vi "Simple SCP File Download.vi"() -> ()   [LabVIEW 2018]
doc: "Downloads, or receives, a relatively small file from a remote SSH server. This is similar to the SCP command line utility when transferring, or copying, a remote file to a local destination. If performance is poor or memory is limited on the local machine, then it could be because the file is relatively large and this implementation is not very efficient for relatively large files."
uses:
  Toolkit/Session/Support/Create from SSH.vi
  Toolkit/Session/Support/Password Authentication.vi
  Toolkit/Channel/Support/Create from SCP Receive.vi
  Toolkit/Channel/Support/Destroy to Session.vi
  Toolkit/Session/Support/Destroy to SSH.vi
  Toolkit/SSH/SSH.lvclass
  Toolkit/Session/Session.lvclass
  Toolkit/Channel/Channel.lvclass
panel:
  in  "Remote File":string
  in  "Local File":path
  in  "Remote SSH Server":string
  in  "Password":string
  in  "Username":string
  # "Overview: Demonstrates transferring, or downloading, a remote file from a SSH server, similar to the SCP command line utility\nInstructions:\n1. Enter the IP address or host name of the remote SSH server. This can be a CompactRIO (cRIO) running the National Instruments Linux Real-Time (NI Linux RT) operating system with the Enable Secure Shell Server (sshd) checkbox checked. \n2. Enter a username. If using a cRIO with a default configuration, then the username is \"admin\".\n3. Enter a password for the username. If using a cRIO with a default configuration, then the password is blank (empty).\n4. Enter the path and/or filename of the remote file to download. Typically, this is a POSIX/UNIX file path with a backslash, \"/\", use to separate directories and the default directory is the remote user's home directory, i.e. \"/home/admin\" on a default configured cRIO.\n5. Select a destination on the local computer for the transfer/download from the remote SSH server.\n6. Run this VI."
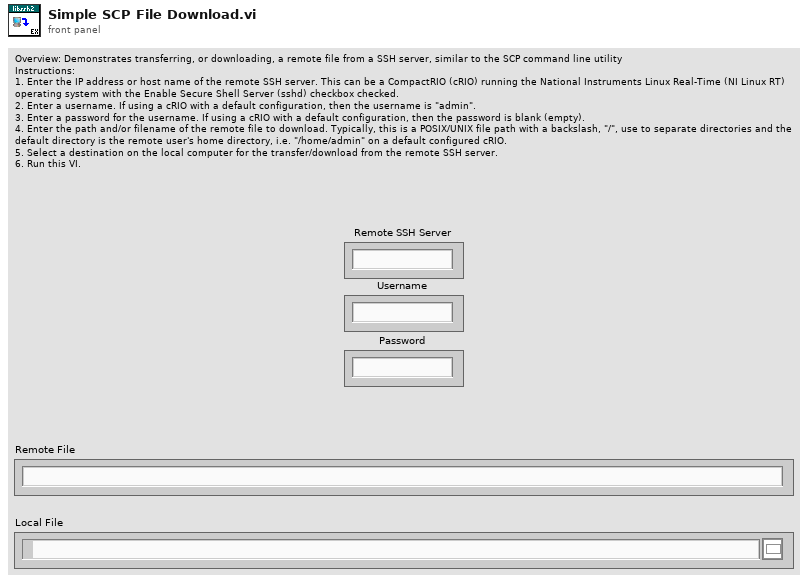
[diagram p1: front panel]
types:
  T1 = enum16{"open", "replace", "create", "open or create", "replace or create", "replace or create with confirmation"}
  T2 = typedef "Toolkit.lvlib/Permissions.ctl" = cluster{"Owner":T3, "Group":T3, "Others":T3}
  T3 = typedef "Toolkit.lvlib/Modes.ctl" = cluster{"Read":bool, "Write":bool, "Execute":bool}
  T4 = cluster{"Access Time":u64, "File Size":u64, "Modified Time":u64, "Permissions":T2}
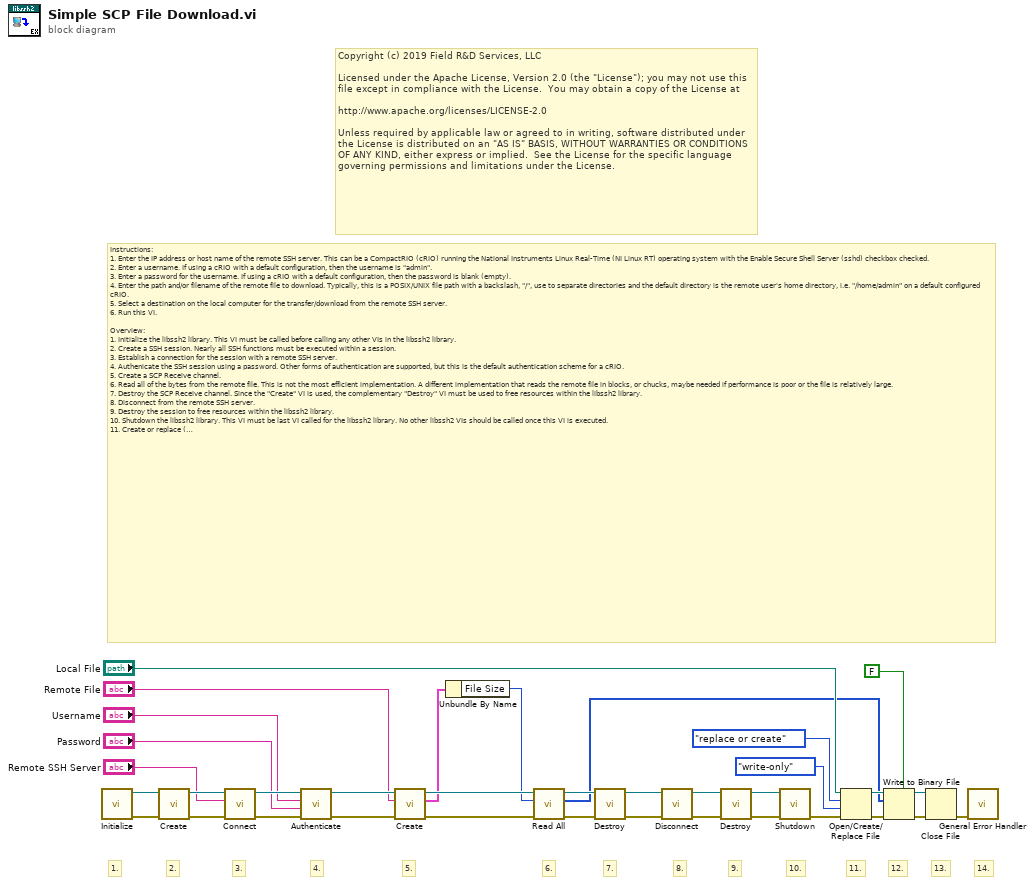
[diagram p0: block diagram]
diagram:
  # "Copyright (c) 2019 Field R&D Services, LLC\n\nLicensed under the Apache License, Version 2.0 (the \"License\"); you may not use this file except in compliance with the License.  You may obtain a copy of the License at\n\nhttp://www.apache.org/licenses/LICENSE-2.0\n\nUnless required by applicable law or agreed to in writing, software distributed under the License is distributed on an \"AS IS\" BASIS, WITHOUT WARRANTIES OR CONDITIONS OF ANY KIND, either express or implied.  See the License for the specific language governing permissions and limitations under the License."
  # "14."
  # "13."
  # "12."
  # "11."
  # "10."
  # "9."
  # "8."
  # "7."
  # "6."
  # "5."
  # "4."
  # "3."
  # "2."
  # "1."
  # "Instructions:\n1. Enter the IP address or host name of the remote SSH server. This can be a CompactRIO (cRIO) running the National Instruments Linux Real-Time (NI Linux RT) operating system with the Enable Secure Shell Server (sshd) checkbox checked. \n2. Enter a username. If using a cRIO with a default configuration, then the username is \"admin\".\n3. Enter a password for the username. If using a cRIO with a default configuration, then the password is blank (empty).\n4. Enter the path and/or filename of the remote file to download. Typically, this is a POSIX/UNIX file path with a backslash, \"/\", use to separate directories and the default directory is the remote user's home directory, i.e. \"/home/admin\" on a default configured cRIO.\n5. Select a destination on the local computer for the transfer/download from the remote SSH server.\n6. Run this VI.\n\nOverview:\n1. Initialize the libssh2 library. This VI must be called before calling any other VIs in the libssh2 library.\n2. Create a SSH session. Nearly all SSH functions must be executed within a session.\n3. Establish a connection for the session with a remote SSH server.\n4. Authenicate the SSH session using a password. Other forms of authentication are supported, but this is the default authentication scheme for a cRIO. \n5. Create a SCP Receive channel.\n6. Read all of the bytes from the remote file. This is not the most efficient implementation. A different implementation that reads the remote file in blocks, or chucks, maybe needed if performance is poor or the file is relatively large.\n7. Destroy the SCP Receive channel. Since the \"Create\" VI is used, the complementary \"Destroy\" VI must be used to free resources within the libssh2 library.\n8. Disconnect from the remote SSH server.\n9. Destroy the session to free resources within the libssh2 library.\n10. Shutdown the libssh2 library. This VI must be last VI called for the libssh2 library. No other libssh2 VIs should be called once this VI is executed.\n11. Create or replace (overwrite) a file to write the read contents from the remote file.\n12. Write the data from the remote file.\n13. Close the file. This is not strictly necessary, but it is good practice.\n14. Provide some error handling and reporting. Libssh2 errors will be in the -8100 range."
  n1 = call "Initialize.vi"() -> ("Error Out"=w22:errorcluster, "SSH"=w21:refnum<class "SSH.lvclass">)  [unwired: 10 in]
  n2 = call-poly "Create.vi"("Error In"=w22, "SSH"=w21) -> ("Error Out"=w34:errorcluster, "Sesssion"=w35:refnum<class "Session.lvclass">)  [unwired: 8 in]
  n3 = call "Connect.vi"("Error In"=w34, "Address"="Remote SSH Server", "Session In"=w35) -> ("Error Out"=w32:errorcluster, "Sesssion Out"=w33:refnum<class "Session.lvclass">)  [unwired: 7 in]
  n4 = call-poly "Authenticate.vi"("Error In"=w32, "Password"="Password", "Username"="Username", "Session In"=w33) -> ("Error Out"=w19:errorcluster, "Sesssion Out"=w20:refnum<class "Session.lvclass">)  [unwired: 6 in]
  n5 = call-poly "Create.vi"("Error In"=w19, "Remote Source Path"="Remote File", "Session"=w20) -> ("Error Out"=w4:errorcluster, "File Information"=w3:T4, "Channel"=w5:refnum<class "Channel.lvclass">)  [unwired: 6 in]
  n6 = Unbundle By Name(w3) -> ("File Size"=w2:u64)
  n7 = call "Read All.vi"("Error In"=w4, "Max Read Size"=w2, "Channel In"=w5) -> ("Error Out"=w9:errorcluster, "Data"=w7:u8[], "Channel Out"=w8:refnum<class "Channel.lvclass">)  [unwired: 5 in, 1 out]
  n8 = call-poly "Destroy.vi"("Error In"=w9, "Channel"=w8) -> ("Error Out"=w27:errorcluster, "Session"=w28:refnum<class "Session.lvclass">)  [unwired: 8 in]
  n9 = call "Disconnect.vi"("Error In"=w27, "Session In"=w28) -> ("Error Out"=w25:errorcluster, "Sesssion Out"=w26:refnum<class "Session.lvclass">)  [unwired: 8 in]
  n10 = call-poly "Destroy.vi"("Error In"=w25, "Session"=w26) -> ("Error Out"=w23:errorcluster, "SSH"=w24:refnum<class "SSH.lvclass">)  [unwired: 8 in]
  n11 = call "Shutdown.vi"("Error In"=w23, "SSH"=w24) -> ("Error Out"=w18:errorcluster)  [unwired: 9 in]
  n12 = Open/Create/Replace File(file path (use dialog)="Local File", error in=w18, operation (0:open)=T1."replace or create", access (0:read/write)=enum16{"read/write", "read-only", "write-only"}."write-only") -> (refnum out=w14:refnum<file>, error out=w13:errorcluster)  [unwired: 2 in, 1 out]
  n13 = Write to Binary File(file (use dialog)=w14, data=w7, error in=w13, 5:FALSE ("prepend array or string size? (T)")) -> (refnum out=w12:refnum<file>, error out=w11:errorcluster)  [unwired: 2 in, 1 out]
  n14 = Close File(refnum=w12, error in=w11) -> (error out=w10:errorcluster)  [unwired: 1 out]
  n15 = call <vilib>:"General Error Handler.vi"("error in (no error)"=w10) -> ()  [unwired: 10 in, 5 out]
